vi "Create Error Object.vi"(8 "error in (no error)":errorcluster) -> (0 "error out":errorcluster, 2 "error":T1)   [LabVIEW 2019, in "JSON-RPC.lvlib"]
uses:
  JSON-RPC.lvlib
  typedefs/Error--Cluster.ctl
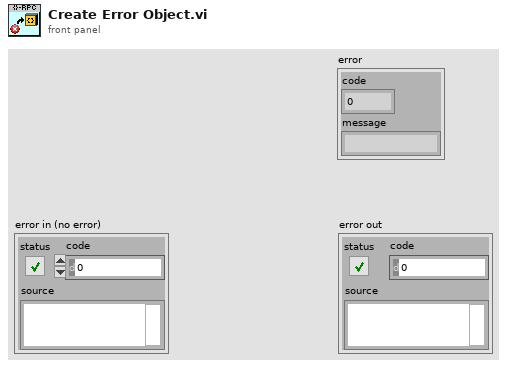
[diagram p1: front panel]
types:
  T1 = typedef "JSON-RPC.lvlib/Error--Cluster.ctl" = cluster{"code":i32, "message":string}
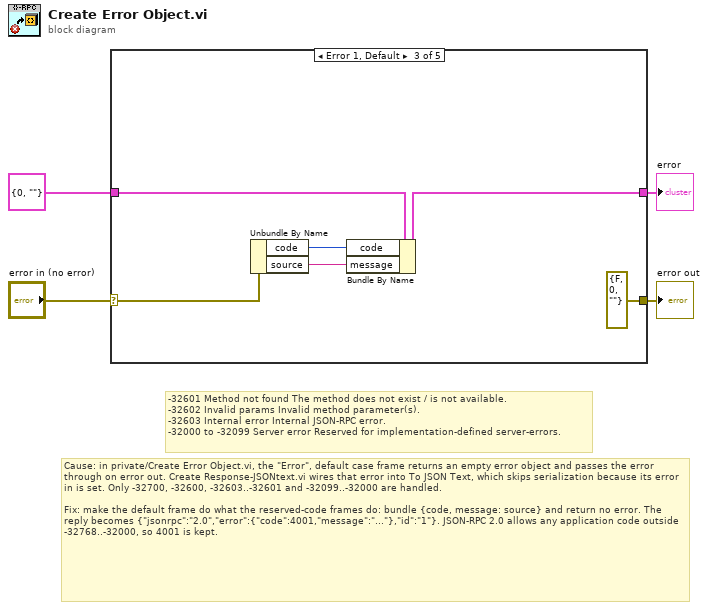
[diagram p0: block diagram]
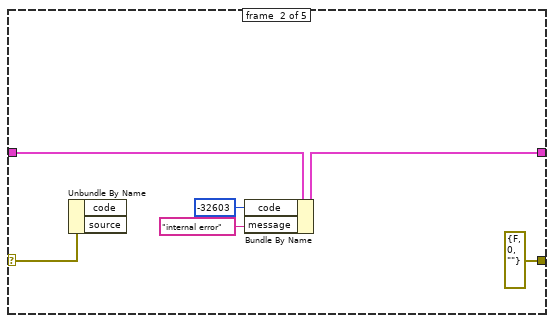
[diagram p3: hidden frame]
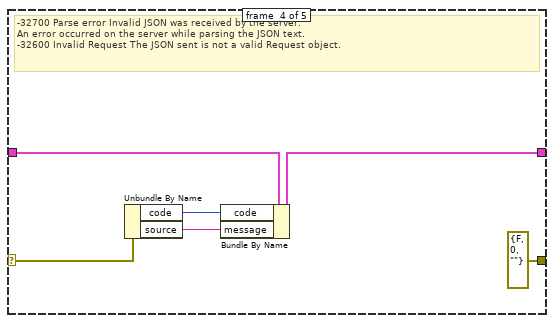
[diagram p4: hidden frame]
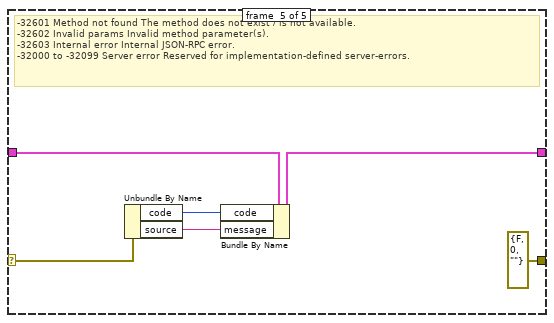
[diagram p5: hidden frame]
diagram:
  # "Cause: in private/Create Error Object.vi, the \"Error\", default case frame returns an empty error object and passes the error through on error out. Create Response-JSONtext.vi wires that error into To JSON Text, which skips serialization because its error in is set. Only -32700, -32600, -32603..-32601 and -32099..-32000 are handled.\n\nFix: make the default frame do what the reserved-code frames do: bundle {code, message: source} and return no error. The reply becomes {\"jsonrpc\":\"2.0\",\"error\":{\"code\":4001,\"message\":\"...\"},\"id\":\"1\"}. JSON-RPC 2.0 allows any application code outside -32768..-32000, so 4001 is kept."
  # "-32601\tMethod not found\tThe method does not exist / is not available.\n-32602\tInvalid params\tInvalid method parameter(s).\n-32603\tInternal error\tInternal JSON-RPC error.\n-32000 to -32099\tServer error\tReserved for implementation-defined server-errors."
  n1 = case shown="Error 1, Default" "error in (no error)" {
    selector: "error in (no error)" -> [w5 w11 w15 w21 w27]
    tunnel: [w5 errorcluster {"status"=FALSE, "code"=0, "source"=""} ("error IO") errorcluster {"status"=FALSE, "code"=0, "source"=""} ("error IO") errorcluster {"status"=FALSE, "code"=0, "source"=""} ("error IO") errorcluster {"status"=FALSE, "code"=0, "source"=""} ("error IO")] -> w3
    tunnel: [_ w9 w13 w19 w25] -> w2
    tunnel: T1 {"code"=0, "message"=""} ("error") -> [_ w10 w14 w18 w24]
    frame #0 {
    }
    frame #1 {
      n2 = Unbundle By Name(w11) -> ()  [unwired: 2 out]
      n3 = Bundle By Name(cluster=w10, "code"=-32603, "message"="internal error") -> (w9:T1)
    }
    frame #2 {
      n4 = Unbundle By Name(w15) -> ("code"=w17:i32, "source"=w16:string)
      n5 = Bundle By Name(cluster=w14, "code"=w17, "message"=w16) -> (w13:T1)
    }
    frame #3 {
      # "-32700\tParse error\tInvalid JSON was received by the server.\nAn error occurred on the server while parsing the JSON text.\n-32600\tInvalid Request\tThe JSON sent is not a valid Request object."
      n6 = Unbundle By Name(w21) -> ("code"=w23:i32, "source"=w22:string)
      n7 = Bundle By Name(cluster=w18, "code"=w23, "message"=w22) -> (w19:T1)
    }
    frame #4 {
      # "-32601\tMethod not found\tThe method does not exist / is not available.\n-32602\tInvalid params\tInvalid method parameter(s).\n-32603\tInternal error\tInternal JSON-RPC error.\n-32000 to -32099\tServer error\tReserved for implementation-defined server-errors."
      n8 = Unbundle By Name(w27) -> ("code"=w29:i32, "source"=w28:string)
      n9 = Bundle By Name(cluster=w24, "code"=w29, "message"=w28) -> (w25:T1)
    }
  }
  "error out" <- w3
  "error" <- w2
